vi "Manipulate Auto Velocities.vi"(8 "Zero Translational V":bool, 9 "Zero V":bool, 10 "Position":cluster{"x":dbl, "y":dbl, "th":dbl}, 11 "Robot Velocities":T2) -> (1 "Done?":bool, 2 "Drive Conditions":T1, 3 "Robot Velocities Out":T2)   [LabVIEW 2023]
uses:
  Robot Global Data.vi
  <vilib>/MRC/MrcLib.lvlib
  swerve-template/Type Definitions/Data/Robot Velocities.ctl
  Drive Conditions.ctl
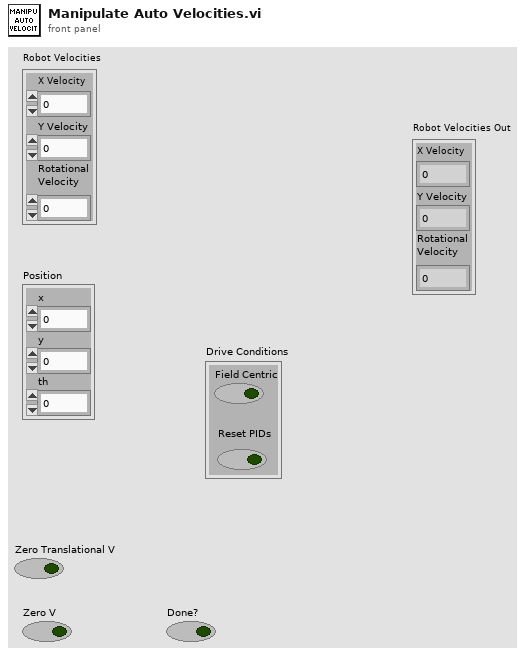
[diagram p1: front panel]
types:
  T1 = typedef "Drive Conditions.ctl" = cluster{"Field Centric":bool, "Reset PIDs":bool}
  T2 = typedef "Robot Velocities.ctl" = cluster{"X Velocity":dbl, "Y Velocity":dbl, "Rotational \nVelocity":dbl}
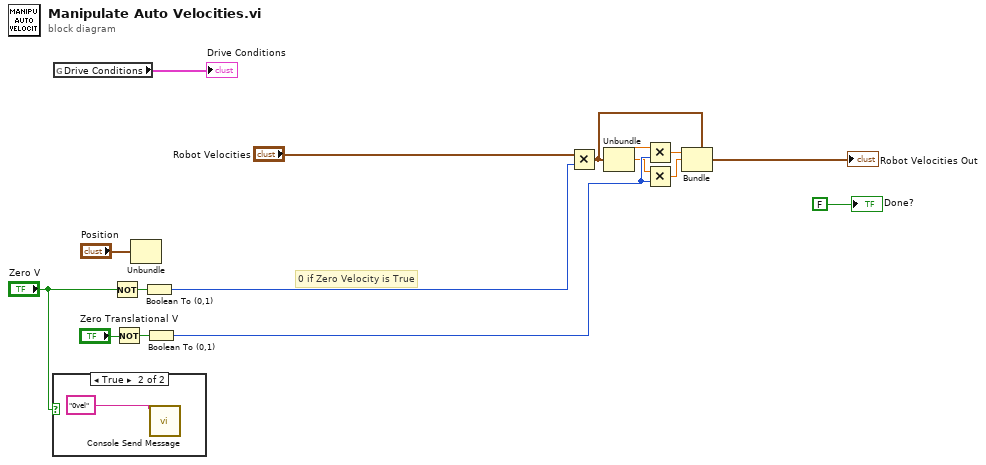
[diagram p0: block diagram]
diagram:
  # "0 if Zero Velocity is True"
  n1 = case shown="True" "Zero V" {
    frame False {
    }
    frame True {
      n2 = call <vilib>:"Console Send Message.vi"("Message"="0vel") -> ()  [unwired: 14 in, 1 out]
    }
  }
  n3 = global read "Robot Global Data.vi" "Drive Conditions"() -> (→"Drive Conditions":cluster{"Field Centric":bool, "Reset PIDs":bool})
  n4 = Not(x="Zero V") -> (.not. x?=w15:bool)
  n5 = Not(x="Zero Translational V") -> (.not. x?=w13:bool)
  n6 = Unbundle("Position") -> ()  [unwired: 3 out]
  n7 = Boolean To (0,1)(Boolean=w15) -> (0, 1=w16:i16)
  n8 = Boolean To (0,1)(Boolean=w13) -> (0, 1=w11:i16)
  n9 = Multiply(x="Robot Velocities", y=w16) -> (x*y=w6:T2)
  n10 = Unbundle(w6) -> ("X Velocity"=w9:dbl, "Y Velocity"=w10:dbl)  [unwired: 1 out]
  n11 = Multiply(x=w9, y=w11) -> (x*y=w8:dbl)
  n12 = Multiply(x=w10, y=w11) -> (x*y=w7:dbl)
  n13 = Bundle(cluster=w6, "X Velocity"=w8, "Y Velocity"=w7) -> (→"Robot Velocities Out":T2)  [unwired: 1 in]
  "Done?" <- FALSE ("Done?")
